vi "YAV_Read.vi"(0 "Device ID":i32, 1 "error in":errorcluster caption="错误输入（无错误）") -> (14 "Light Voltage (V)":dbl, 15 "DI0 Raw":bool, 16 "DI1 Raw":bool, 17 "Tilt":bool, 18 "Motion":bool, 19 "error out":errorcluster caption="错误输出")   [LabVIEW 2020]
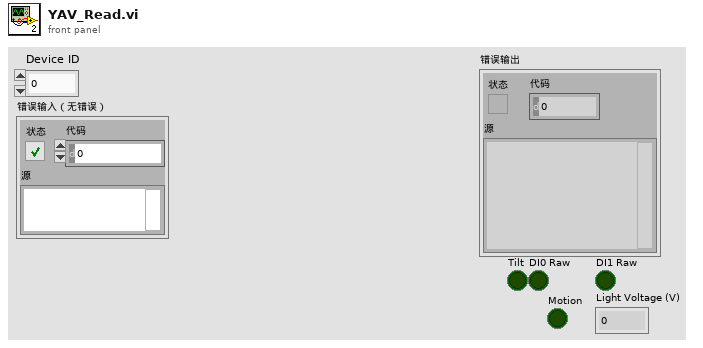
[diagram p1: front panel]
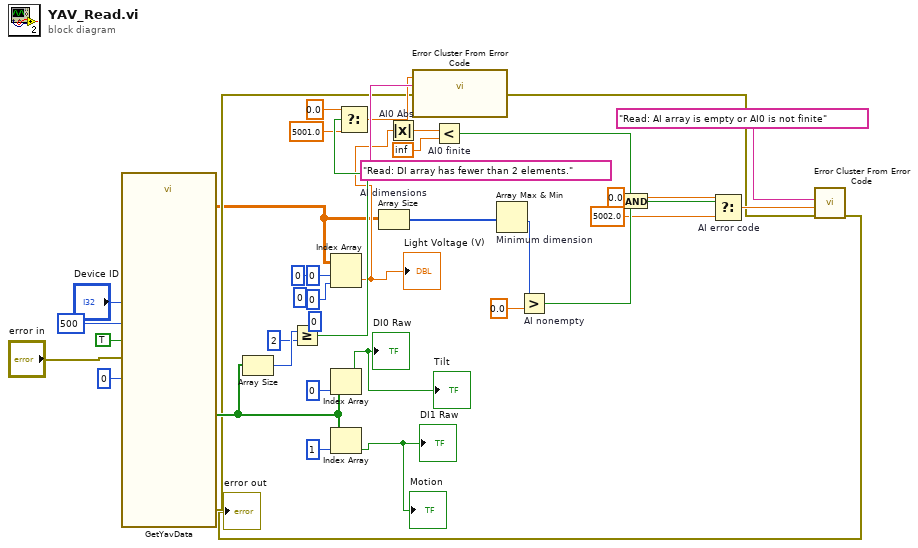
[diagram p0: block diagram]
diagram:
  (unwired) 0 ("索引 (列)")
  (unwired) 0 ("索引 (行)")
  (unwired) 0 ("索引 (行)")
  n1 = call "GetYavData.vi"("ID"="Device ID", "第一量程通道数"=u8 0, "初始化"=TRUE, "采样长度"=500, "错误输入（无错误）"="error in") -> ("DI"=w26:bool[], "数组 列通道号"=w4:dbl[][], "error out"=w18:errorcluster)  [unwired: 2 in, 10 out]
  n2 = Array Size(array=w26) -> (size(s)=w25:i32)
  n3 = Greater Or Equal?(x=w25, y=2) -> (x >= y?=w23:bool)
  n4 = Index Array(array=w4, index (row)=0 ("禁用的索引 (行)"), index (col)=0 ("禁用的索引 (列)")) -> (element=w5:dbl)
  "Light Voltage (V)" <- w5
  n5 = Index Array(array=w26, index=0 ("索引")) -> (element=→"Tilt" →"DI0 Raw":bool)
  n6 = Index Array(array=w26, index=1 ("索引")) -> (element=→"DI1 Raw" →"Motion":bool)
  n7 = Select(t=0.0, s=w23, f=5001.0) -> (s? t:f=w19:dbl)
  n8 = Array Size "AI dimensions"(array=w4) -> (size(s)=w16:i32[])
  n9 = Absolute Value "AI0 Abs"(x=w5) -> (abs(x)=w17:dbl)
  n10 = call <vilib>:"Error Cluster From Error Code.vi"("error in (no error)"=w18, "error message (\"\")"="Read: DI array has fewer than 2 elements." ("error message (\"\")"), "error code (0)"=w19) -> ("error out"=w3:errorcluster)  [unwired: 6 in]
  n11 = Less? "AI0 finite"(x=w17, y=inf) -> (x < y?=w13:bool)
  n12 = Array Max & Min "Minimum dimension"(array=w16) -> (min value=w15:i32)  [unwired: 3 out]
  n13 = Greater? "AI nonempty"(x=w15, y=0.0) -> (0:w12:bool)
  n14 = And(x=w13, y=w12) -> (x .and. y?=w11:bool)
  n15 = Select "AI error code"(t=0.0, s=w11, f=5002.0) -> (s? t:f=w8:dbl)
  n16 = call <vilib>:"Error Cluster From Error Code.vi"("error in (no error)"=w3, "error message (\"\")"="Read: AI array is empty or AI0 is not finite" ("error message (\"\")"), "error code (0)"=w8) -> ("error out"=→"error out":errorcluster)  [unwired: 6 in]
